vi "Build Help Info for Help Items.vi"(5 "Subfolder":string, 6 "CHM Tag mode":enum16{"HTML Filename", "Index Keyword"}(ring), 7 "Help Targeting":T2(ring)=enum."relative", 8 "error in":errorcluster, 10 "CHM File (empty)":path, 11 "Help Items":T3(array[cluster])) -> (0 "error out":errorcluster, 2 "Source Files Help Info":T1(array[cluster]), 3 "Source File Paths":path[](array[path]))   [LabVIEW 2014, in "VIHelpeksAPI.lvlib"]
doc: "The VI prepares information for linking VIs and palettes to help files. The input for this VI can be read from the <b>Help Info File</b> created by VI Helpeks during help generation.\n\nThe <b>Example VI</b> demonstrating the use of VIHelpeks API can be opened using the \"Tools >> VI Helpeks >> Help and Support\" menu. Alternatively, you can launch the <b>NI Example Finder</b> and search for \"VI Helpeks\", or find it within the <b><labview>\\Examples\\VI Helpeks</b> folder.\n\n::: VI Helpeks :::\nCopyright (c) 2000-2026 Konstantin Shifershteyn. All rights reserved."
uses:
  VIHelpeksAPI.lvlib
panel:
  # "VI Helpeks\nCopyright (c) 2012-2026 Konstantin Shifershteyn"
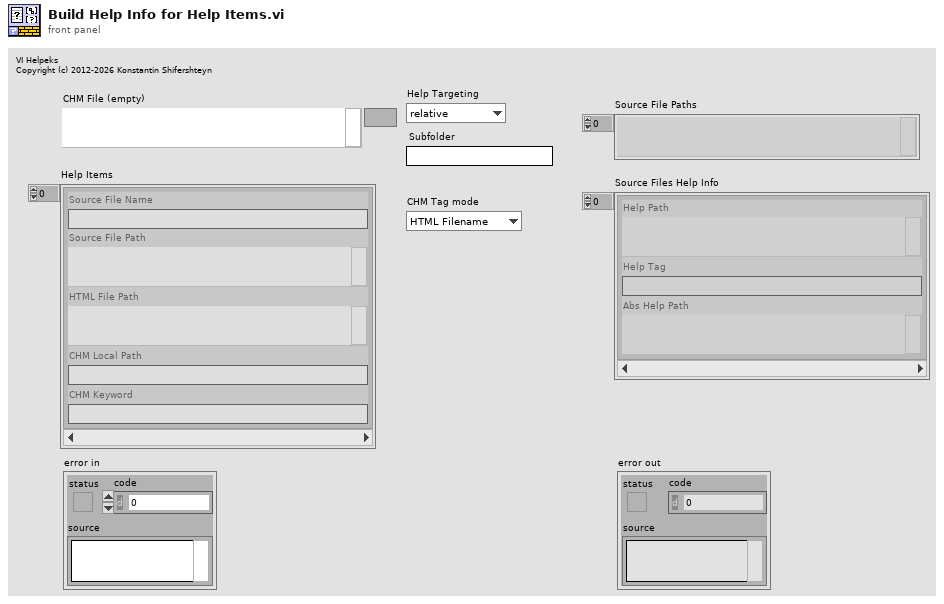
[diagram p1: front panel]
types:
  T1 = cluster{"Help Path":path, "Help Tag":string, "Abs Help Path":path}[]
  T2 = enum16{"absolute", "relative", "<helpdir>", "<userlib>", "<vilib>", "<instrlib>"}
  T3 = cluster{"Source File Name":string, "Source File Path":path, "HTML File Path":path, "CHM Local Path":string, "CHM Keyword":string}[]
  T4 = cluster{"Help Path":path, "Help Tag":string, "Abs Help Path":path}
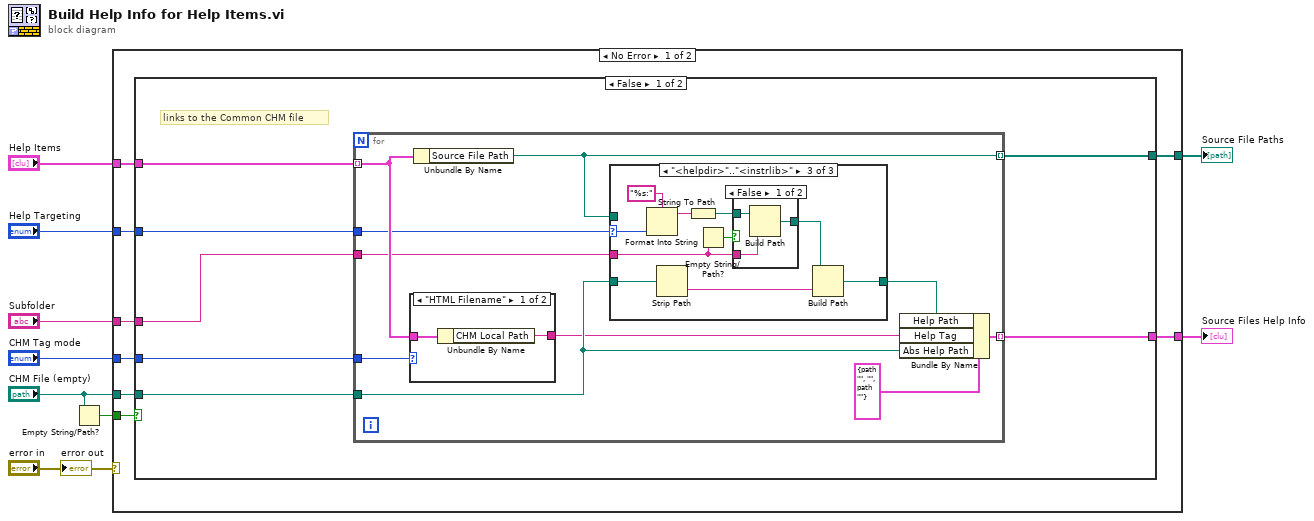
[diagram p0: block diagram]
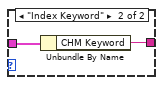
[diagram p2: hidden frame]
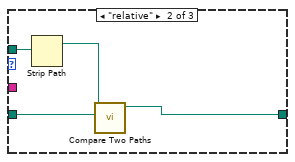
[diagram p4: hidden frame]
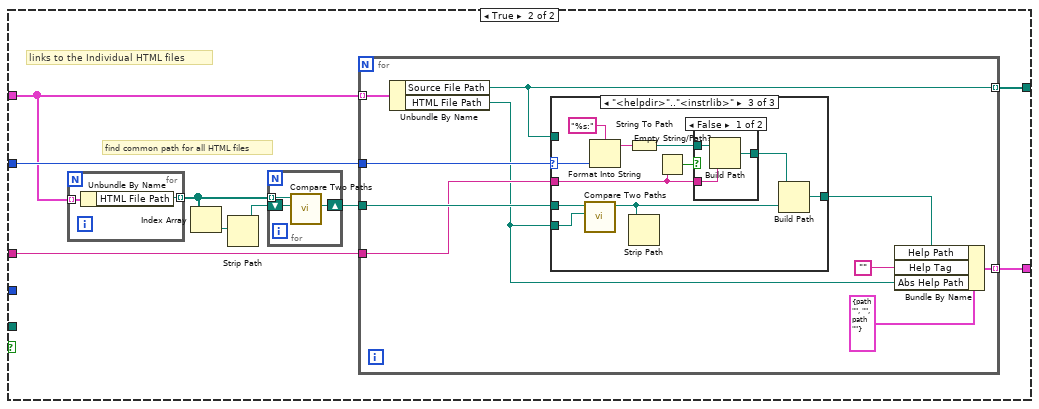
[diagram p6: hidden frame]
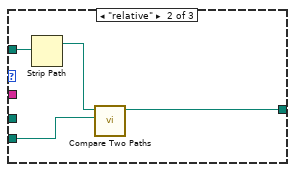
[diagram p8: hidden frame]
diagram:
  n1 = Empty String/Path?(string/path="CHM File (empty)") -> (empty?=w1:bool)
  n2 = case shown="No Error" "error in" {
    tunnel: "CHM Tag mode" -> [w17 _]
    tunnel: "Help Targeting" -> [w16 _]
    tunnel: "Help Items" -> [w15 _]
    tunnel: "CHM File (empty)" -> [w14 _]
    tunnel: "Subfolder" -> [w13 _]
    tunnel: [w12 _] -> w5
    tunnel: [w11 _] -> w4
    tunnel: w1 -> [w10 _]
    frame No Error {
      n3 = case shown="False" w10 {
        tunnel: w17 -> [w24 _]
        tunnel: w16 -> [w23 w66]
        tunnel: w15 -> [w22 w65]
        tunnel: w14 -> [w21 _]
        tunnel: w13 -> [w20 w63]
        tunnel: [w19 w62] -> w12
        tunnel: [w18 w61] -> w11
        frame False {
          # "links to the Common CHM file"
          n4 = for {
            tunnel: w22 -> [w32] mode=indexing
            tunnel: w21 -> [w34]
            tunnel: w24 -> [w33]
            tunnel: [w30] -> w19 mode=indexing
            tunnel: w23 -> [w29]
            tunnel: w20 -> [w27]
            tunnel: [w26] -> w18 mode=indexing
            n5 = case shown="\"HTML Filename\"" w33 {
              tunnel: w32 -> [w36 w38]
              tunnel: [w35 w37] -> w31
              frame "HTML Filename" {
                n6 = Unbundle By Name(w36) -> ("CHM Local Path"=w35:string)
              }
              frame "Index Keyword" {
                n7 = Unbundle By Name(w38) -> ("CHM Keyword"=w37:string)
              }
            }
            n8 = Unbundle By Name(w32) -> ("Source File Path"=w26:path)
            n9 = case shown="\"<helpdir>\"..\"<instrlib>\"" w29 {
              selector: w29 -> [_ _ w51]
              tunnel: [w39 w42 w53] -> w28
              tunnel: w34 -> [w39 w43 w45]
              tunnel: w27 -> [_ _ w46]
              tunnel: w26 -> [_ w41 _]
              frame "absolute" {
              }
              frame "relative" {
                n10 = Strip Path(path=w41) -> (stripped path=w40:path)  [unwired: 1 out]
                n11 = call <vilib>:"Compare Two Paths.vi"("Path 2"=w43, "Path 1"=w40) -> ("Relative Path from 1 to 2"=w42:path)  [unwired: 6 in, 3 out]
              }
              frame "<helpdir>".."<instrlib>" {
                n12 = Format Into String(format string="%s:", w51) -> (resulting string=w50:string)  [unwired: 2 in, 1 out]
                n13 = Strip Path(path=w45) -> (name=w44:string)  [unwired: 1 out]
                n14 = String To Path(string=w50) -> (path=w49:path)
                n15 = Empty String/Path?(string/path=w46) -> (empty?=w47:bool)
                n16 = case shown="False" w47 {
                  tunnel: w49 -> [w56 w57]
                  tunnel: [w55 w57] -> w48
                  tunnel: w46 -> [w54 _]
                  frame False {
                    n17 = Build Path(base path=w56, name or relative path=w54) -> (appended path=w55:path)
                  }
                  frame True {
                  }
                }
                n18 = Build Path(base path=w48, name or relative path=w44) -> (appended path=w53:path)
              }
            }
            n19 = Bundle By Name(cluster=T4 {"Help Path"=path "", "Help Tag"="", "Abs Help Path"=path ""} ("Help Item Info"), "Help Path"=w28, "Help Tag"=w31, "Abs Help Path"=w34) -> (w30:T4)
          }
        }
        frame True {
          # "find common path for all HTML files"
          # "links to the Individual HTML files"
          n20 = for {
            tunnel: w65 -> [w71] mode=indexing
            tunnel: [w70] -> w60 mode=indexing
            n21 = Unbundle By Name(w71) -> ("HTML File Path"=w70:path)
          }
          n22 = Index Array(array=w60) -> (element=w59:path)  [unwired: 1 in]
          n23 = Strip Path(path=w59) -> (stripped path=w58:path)  [unwired: 1 out]
          n24 = for {
            shift-right: [w69] -> w64
            shift-left: w58 -> [w68]
            tunnel: w60 -> [w67] mode=indexing
            n25 = call <vilib>:"Compare Two Paths.vi"("Path 2"=w68, "Path 1"=w67) -> ("Common Path"=w69:path)  [unwired: 6 in, 3 out]
          }
          n26 = for {
            tunnel: w65 -> [w81] mode=indexing
            tunnel: [w80] -> w62 mode=indexing
            tunnel: w66 -> [w79]
            tunnel: w64 -> [w77]
            tunnel: w63 -> [w76]
            tunnel: [w75] -> w61 mode=indexing
            n27 = Unbundle By Name(w81) -> ("Source File Path"=w75:path, "HTML File Path"=w72:path)
            n28 = case shown="\"<helpdir>\"..\"<instrlib>\"" w79 {
              selector: w79 -> [_ _ w93]
              tunnel: [w82 w85 w97] -> w78
              tunnel: w72 -> [w82 w86 w95]
              tunnel: w77 -> [_ _ w96]
              tunnel: w76 -> [_ _ w88]
              tunnel: w75 -> [_ w84 _]
              frame "absolute" {
              }
              frame "relative" {
                n29 = Strip Path(path=w84) -> (stripped path=w83:path)  [unwired: 1 out]
                n30 = call <vilib>:"Compare Two Paths.vi"("Path 2"=w86, "Path 1"=w83) -> ("Relative Path from 1 to 2"=w85:path)  [unwired: 6 in, 3 out]
              }
              frame "<helpdir>".."<instrlib>" {
                n31 = call <vilib>:"Compare Two Paths.vi"("Path 2"=w95, "Path 1"=w96) -> ("Relative Path from 1 to 2"=w87:path)  [unwired: 6 in, 3 out]
                n32 = Format Into String(format string="%s:", w93) -> (resulting string=w92:string)  [unwired: 2 in, 1 out]
                n33 = String To Path(string=w92) -> (path=w91:path)
                n34 = Strip Path(path=w87) -> ()  [unwired: 2 out]
                n35 = Empty String/Path?(string/path=w88) -> (empty?=w89:bool)
                n36 = case shown="False" w89 {
                  tunnel: w91 -> [w100 w101]
                  tunnel: [w99 w101] -> w90
                  tunnel: w88 -> [w98 _]
                  frame False {
                    n37 = Build Path(base path=w100, name or relative path=w98) -> (appended path=w99:path)
                  }
                  frame True {
                  }
                }
                n38 = Build Path(base path=w90, name or relative path=w87) -> (appended path=w97:path)
              }
            }
            n39 = Bundle By Name(cluster=T4 {"Help Path"=path "", "Help Tag"="", "Abs Help Path"=path ""} ("Help Item Info"), "Help Path"=w78, "Help Tag"="", "Abs Help Path"=w72) -> (w80:T4)
          }
        }
      }
    }
    frame Error {
    }
  }
  "Source Files Help Info" <- w5
  "Source File Paths" <- w4
  "error out" <- "error in"
